vi "Deploy.vi"() -> ()   [LabVIEW 2023]
doc: "Tools >> Systemcore >> Deploy: saves the project's modified VIs, commits the project and deploys it, with the add-ons it uses, to the robot in systemcore.ini."
panel:
  out "Status":string
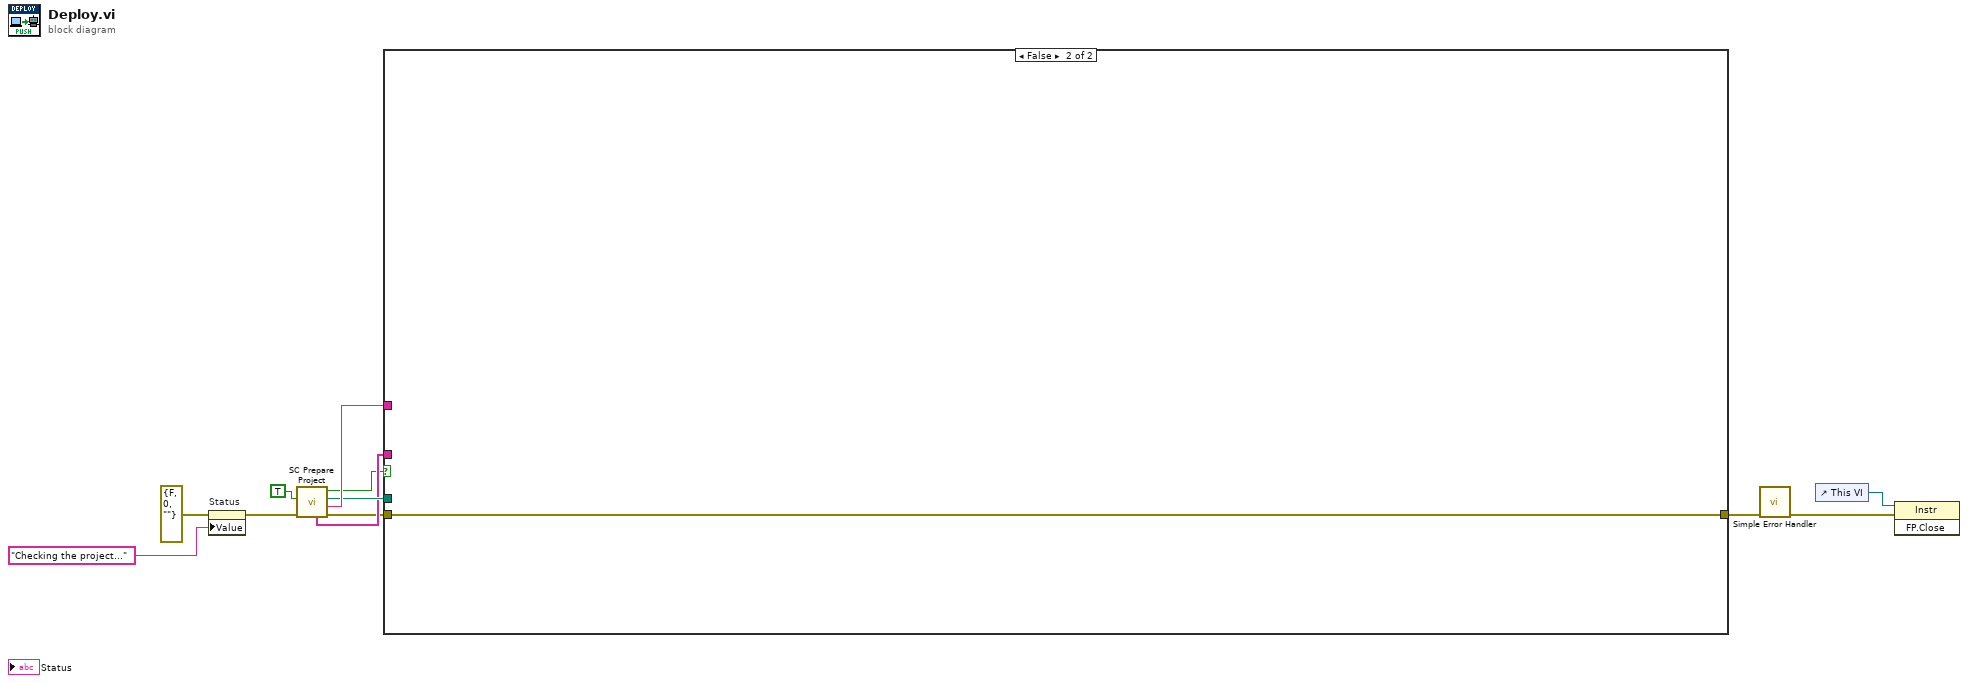
[diagram p0: block diagram]
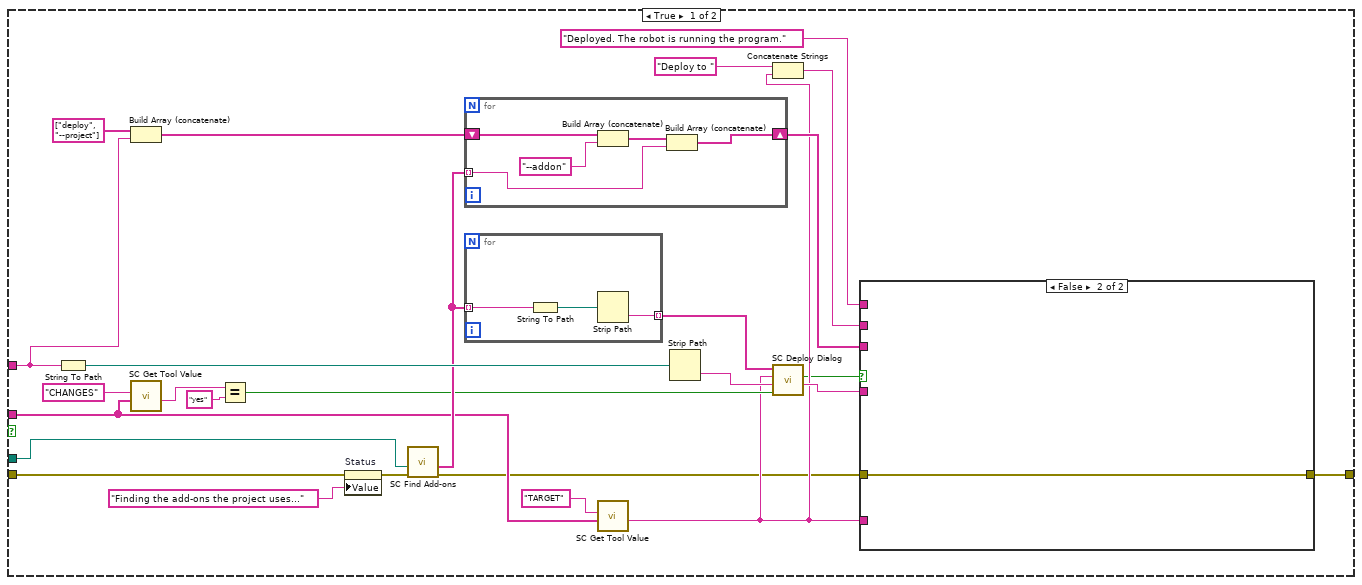
[diagram p2: hidden frame]
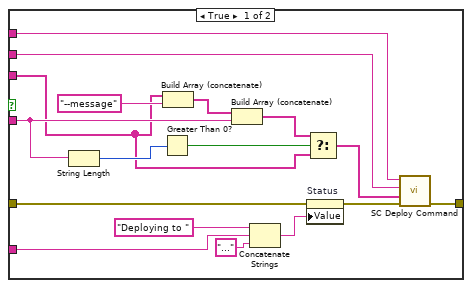
[diagram p3: hidden frame]
diagram:
  n1 = property on="Status" class="Str"(error in=errorcluster {"status"=FALSE, "code"=0, "source"=""}, "Value"="Checking the project...") -> (error out=w9:errorcluster)  [unwired: 1 in, 1 out]
  n2 = call "SC Prepare Project.vi"("error in (no error)"=w9, "save VIs?"=TRUE) -> ("error out"=w5:errorcluster, "project root"=w8:string, "entry VI"=w7:path, "ready?"=w4:bool, "tool lines"=w6:string[])  [unwired: 5 in]
  n3 = case shown="False" w4 {
    tunnel: w8 -> [w30 _]
    tunnel: w7 -> [w36 _]
    tunnel: w6 -> [w27 _]
    tunnel: w5 -> [w38 w65]
    tunnel: [w13 w65] -> w3
    frame True {
      n4 = String To Path(string=w30) -> (path=w29:path)
      n5 = Build Array (concatenate)(string[] ["deploy", "--project"], w30) -> (w33:string[])
      n6 = call "SC Get Tool Value.vi"("tool lines"=w27, "key"="CHANGES") -> ("value"=w25:string)  [unwired: 8 in, 1 out]
      n7 = Equal?(x=w25, y="yes") -> (x = y?=w21:bool)
      n8 = property on="Status" class="Str"(error in=w38, "Value"="Finding the add-ons the project uses...") -> (error out=w35:errorcluster)  [unwired: 1 in, 1 out]
      n9 = call "SC Find Add-ons.vi"("error in (no error)"=w35, "entry VI"=w36) -> ("error out"=w15:errorcluster, "add-on directories"=w28:string[])  [unwired: 8 in]
      n10 = for {
        tunnel: w28 -> [w61] mode=indexing
        shift-right: [w60] -> w20
        shift-left: w33 -> [w64]
        n11 = Build Array (concatenate)(w64, "--addon") -> (w62:string[])
        n12 = Build Array (concatenate)(w62, w61) -> (w60:string[])
      }
      n13 = for {
        tunnel: w28 -> [w59] mode=indexing
        tunnel: [w57] -> w22 mode=indexing
        n14 = String To Path(string=w59) -> (path=w58:path)
        n15 = Strip Path(path=w58) -> (name=w57:string)  [unwired: 1 out]
      }
      n16 = call "SC Get Tool Value.vi"("tool lines"=w27, "key"="TARGET") -> ("value"=w18:string)  [unwired: 8 in, 1 out]
      n17 = Strip Path(path=w29) -> (name=w23:string)  [unwired: 1 out]
      n18 = Concatenate Strings("Deploy to ", w18) -> (w17:string)
      n19 = call "SC Deploy Dialog.vi"("changes?"=w21, "project"=w23, "robot"=w18, "add-ons"=w22) -> ("message"=w19:string, "deploy?"=w14:bool)  [unwired: 6 in]
      n20 = case shown="False" w14 {
        tunnel: w20 -> [w49 _]
        tunnel: w19 -> [w53 _]
        tunnel: w18 -> [w47 _]
        tunnel: w17 -> [w42 _]
        tunnel: "Deployed. The robot is running the program." -> [w41 _]
        tunnel: w15 -> [w45 w56]
        tunnel: [w39 w56] -> w13
        frame True {
          n21 = String Length(string=w53) -> (length=w52:i32)
          n22 = Greater Than 0?(x=w52) -> (x > 0?=w51:bool)
          n23 = Build Array (concatenate)(w49, "--message") -> (w54:string[])
          n24 = Build Array (concatenate)(w54, w53) -> (w50:string[])
          n25 = Concatenate Strings("Deploying to ", w47, "...") -> (w44:string)
          n26 = property on="Status" class="Str"(error in=w45, "Value"=w44) -> (error out=w40:errorcluster)  [unwired: 1 in, 1 out]
          n27 = Select(t=w50, s=w51, f=w49) -> (s? t:f=w43:string[])
          n28 = call "SC Deploy Command.vi"("error in (no error)"=w40, "arguments"=w43, "title"=w42, "OK message"=w41) -> ("error out"=w39:errorcluster)  [unwired: 6 in, 1 out]
        }
        frame False {
        }
      }
    }
    frame False {
    }
  }
  n29 = call <vilib>:"Simple Error Handler.vi"("error in (no error)"=w3) -> ("error out"=w1:errorcluster)  [unwired: 4 in, 4 out]
  n30 = control-ref of="This VI"() -> (w2:refnum<vi>)
  n31 = invoke class="Instr" method="FP.Close"(reference=w2, error in=w1) -> ()  [unwired: 1 in, 3 out]
